vi "onExecuteJob.vi"(8 "error in (no error)":errorcluster, 10 "stdin":string, 11 "Job.StaticVIRef in":refnum<class "Job.StaticVIRef.lvclass">) -> (0 "error out":errorcluster, 1 "exception":i32, 2 "stdout":string, 3 "Job.StaticVIRef out":refnum<class "Job.StaticVIRef.lvclass">)   [LabVIEW 2013, in "openCronJob.lvlib" / "Job.StaticVIRef.lvclass"]
uses:
  Job.StaticVIRef.lvclass
  Job.StaticVIRef.lvclass/Job.StaticVIRef.ctl
panel:
  # "RUNNING A JOB"
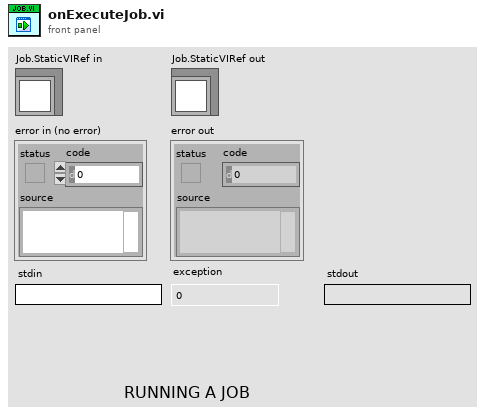
[diagram p1: front panel]
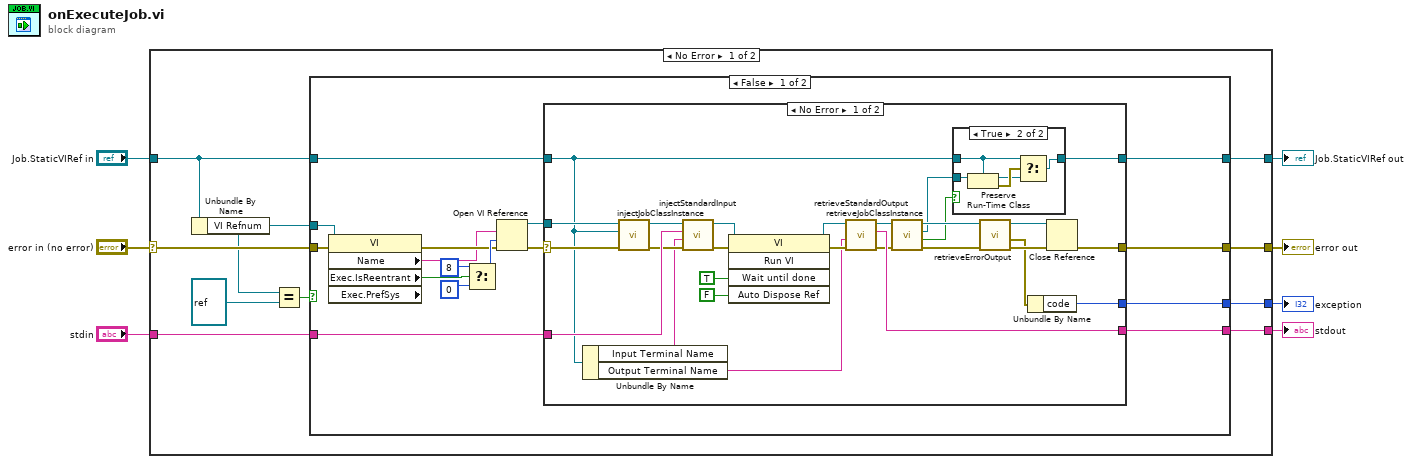
[diagram p0: block diagram]
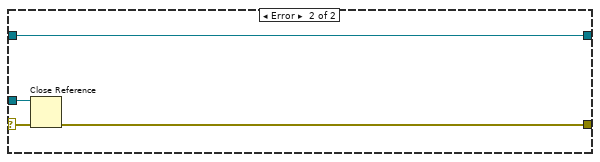
[diagram p3: hidden frame]
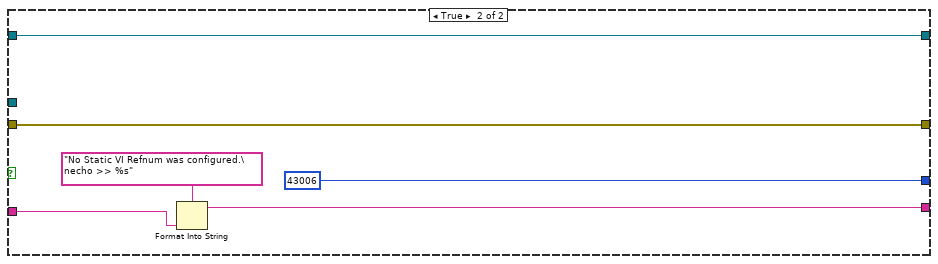
[diagram p4: hidden frame]
diagram:
  n1 = case shown="No Error" "error in (no error)" {
    selector: "error in (no error)" -> [w13 w78]
    tunnel: "stdin" -> [w17 _]
    tunnel: "Job.StaticVIRef in" -> [w8 w77]
    tunnel: [w16 _] -> w5
    tunnel: [w15 w78] -> w4
    tunnel: [w14 _] -> w3
    tunnel: [w9 w77] -> w1
    frame No Error {
      n2 = Unbundle By Name(w8) -> ("VI Refnum"=w12:refnum<vi>)
      n3 = Equal?(x=w12, y=refnum<vi> refnum) -> (x = y?=w10:bool)
      n4 = case shown="False" w10 {
        tunnel: w17 -> [w33 w75]
        tunnel: [w32 w74] -> w16
        tunnel: [w31 w73] -> w15
        tunnel: [w18 43006 ("exception")] -> w14
        tunnel: w13 -> [w23 w73]
        tunnel: w12 -> [w30 _]
        tunnel: [w19 w71] -> w9
        tunnel: w8 -> [w20 w71]
        frame False {
          n5 = property class="VI" props=["Name", "Exec.IsReentrant", "Exec.PrefSys"](reference=w30, error in=w23) -> (error out=w22:errorcluster, "Name"=w21:string, "Exec.IsReentrant"=w28:bool)  [unwired: 2 out]
          n6 = Select(t=8 ("options"), s=w28, f=0 ("options")) -> (s? t:f=w26:i32)
          n7 = Open VI Reference(vi path=w21, options=w26, error in (no error)=w22) -> (vi reference=w25:refnum<vi>, error out=w24:errorcluster)  [unwired: 3 in]
          n8 = case shown="No Error" w24 {
            selector: w24 -> [w48 w68]
            tunnel: w33 -> [w58 _]
            tunnel: [w56 _] -> w32
            tunnel: [w52 w69] -> w31
            tunnel: w25 -> [w51 w70]
            tunnel: w20 -> [w35 w67]
            tunnel: [w36 w67] -> w19
            tunnel: [w42 _] -> w18
            frame No Error {
              n9 = Unbundle By Name(w35) -> ("Input Terminal Name"=w45:string, "Output Terminal Name"=w47:string)
              n10 = call "injectJobClassInstance.vi"("error in (no error)"=w48, "Job"=w35, "VI in"=w51) -> ("error out"=w49:errorcluster, "VI out"=w50:refnum<vi>)  [unwired: 7 in]
              n11 = call "injectStandardInput.vi"("error in (no error)"=w49, "control name (stdin)"=w45, "stdin"=w58, "VI in"=w50) -> ("error out"=w54:errorcluster, "VI out"=w57:refnum<vi>)  [unwired: 6 in]
              n12 = invoke class="VI" method="Run VI"(reference=w57, error in=w54, "Wait until done"=TRUE ("Wait Until Done"), "Auto Dispose Ref"=FALSE ("Auto Dispose Reference")) -> (reference out=w46:refnum<vi>, error out=w55:errorcluster)  [unwired: 1 in, 3 out]
              n13 = call "retrieveStandardOutput.vi"("error in (no error)"=w55, "control name (stdout)"=w47, "VI in"=w46) -> ("error out"=w39:errorcluster, "stdout"=w56:string, "VI out"=w41:refnum<vi>)  [unwired: 6 in]
              n14 = call "retrieveJobClassInstance.vi"("error in (no error)"=w39, "VI in"=w41) -> ("error out"=w38:errorcluster, "found"=w37:bool, "Job"=w34:refnum<class "Job.lvclass">, "VI out"=w40:refnum<vi>)  [unwired: 6 in]
              n15 = case shown="True" w37 {
                tunnel: [w61 w62] -> w36
                tunnel: w35 -> [w61 w64]
                tunnel: w34 -> [_ w66]
                frame False {
                }
                frame True {
                  n16 = Preserve Run-Time Class(object in=w66, 2:w64) -> (object out=w63:refnum<class "Job.StaticVIRef.lvclass">, error out=w65:errorcluster)  [unwired: 1 in]
                  n17 = Select(t=w64, s=w65, f=w63) -> (s? t:f=w62:refnum<class "Job.StaticVIRef.lvclass">)
                }
              }
              n18 = call "retrieveErrorOutput.vi"("error in (no error)"=w38, "VI in"=w40) -> ("error out"=w44:errorcluster, "VI Error Out"=w43:errorcluster, "VI out"=w53:refnum<vi>)  [unwired: 7 in]
              n19 = Unbundle By Name(w43) -> ("code"=w42:i32)
              n20 = Close Reference(reference=w53, error in (no error)=w44) -> (error out=w52:errorcluster)
            }
            frame Error {
              n21 = Close Reference(reference=w70, error in (no error)=w68) -> (error out=w69:errorcluster)
            }
          }
        }
        frame True {
          n22 = Format Into String(format string="No Static VI Refnum was configured.\necho >> %s", w75) -> (resulting string=w74:string)  [unwired: 2 in, 1 out]
        }
      }
    }
    frame Error {
    }
  }
  "error out" <- w4
  "Job.StaticVIRef out" <- w1
  "exception" <- w3
  "stdout" <- w5
